vi "Lua Dispose.vi"(8 "error in (no error)":errorcluster, 11 "Lua in":refnum<class "Lua.lvclass">) -> (0 "error out":errorcluster)   [LabVIEW 2020, in "Lua for LabVIEW.lvlib" / "Lua.lvclass"]
uses:
  Lua.lvclass
  Lua.lvclass/Lua.ctl
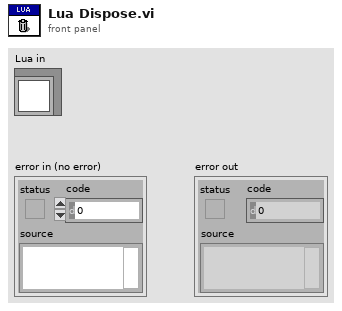
[diagram p1: front panel]
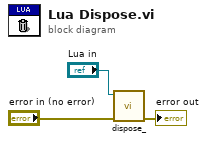
[diagram p0: block diagram]
diagram:
  n1 = call-dynamic "dispose_.vi"("error in (no error)"="error in (no error)", "Lua in"="Lua in") -> ("error out"=→"error out":errorcluster)  [unwired: 9 in]
